vi "VM - Type Code to CalcExpress Data Type.vi"(11 "type code (1)":u32=1) -> (3 "CalcExpress Data Type":T1=enum."DBL Number")   [LabVIEW 2021]
doc: "The VI converts a numeric datatype code to CalcExpress Data Type enum.\n\n::: CalcExpress Toolkit :::\nCopyright (c) 2000-2026 Konstantin Shifershteyn. All rights reserved."
uses:
  cetypes.llb/CalcExpress Data Type.ctl
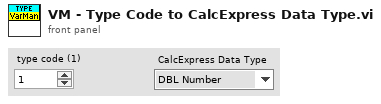
[diagram p1: front panel]
types:
  T1 = typedef "CalcExpress Data Type.ctl" = enum32{"String", "DBL Number", "identifier", "1D Array of DBL", "2D Array of DBL", "CDB Number", "1D Array of CDB", "2D Array of CDB", "1D Array of String", "2D Array of String", "Unknown data type"}
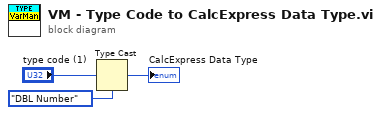
[diagram p0: block diagram]
diagram:
  n1 = Type Cast(type=CalcExpress_Data_Type."DBL Number" ("data type"), x="type code (1)") -> (*(type *) &x=→"CalcExpress Data Type":T1)
